vi "setUp.vi"(8 "error in (no error)":errorcluster) -> (0 "error out":errorcluster, 2 "connection ID":refnum<k5>, 3 "session":T1)   [LabVIEW 2017, in "support.lvlib"]
doc: "Initialize the library, open a connection and authenticate a session with the SSH server."
uses:
  support.lvlib
  libssh2/Session Refnum.ctl
  <vilib>/Utility/error.llb/DialogType.ctl
  libssh2/libssh2_session_handshake_tcp.vi
  libssh2/libssh2_init_default.vi
  libssh2/libssh2_session_init_ex.vi
  <vilib>/Utility/tcp.llb/TCP Get Raw Net Object.vi
  libssh2/libssh2_session_handshake_socket.vi
  libssh2/libssh2.lvlib
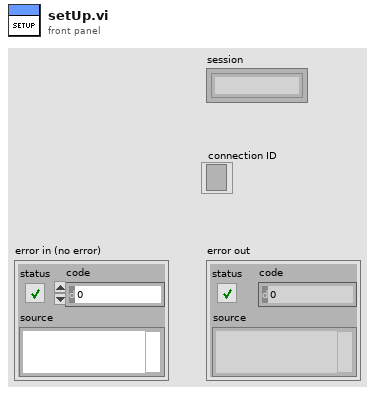
[diagram p1: front panel]
types:
  T1 = typedef "libssh2.lvlib/Session Refnum.ctl" = refnum<k1>
  T2 = typedef "DialogType.ctl" = u16
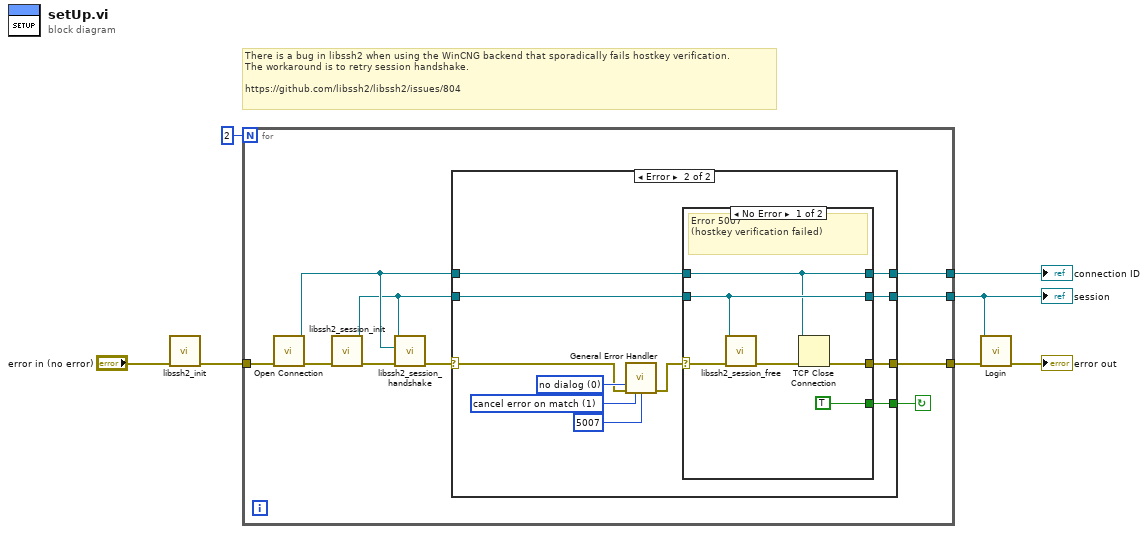
[diagram p0: block diagram]
diagram:
  # "There is a bug in libssh2 when using the WinCNG backend that sporadically fails hostkey verification.\nThe workaround is to retry session handshake.\n\nhttps://github.com/libssh2/libssh2/issues/804"
  n1 = call-poly "libssh2_init.vi"("error in (no error)"="error in (no error)") -> ("error out"=w7:errorcluster)  [unwired: 10 in]
  n2 = for {
    N: 2 -> [_]
    tunnel: w7 -> [w16]
    tunnel: [w13] -> w4
    tunnel: [w11] -> w3
    tunnel: [w9] -> w2
    stop <- w8 continue-if-true
    n3 = call "Open Connection.vi"("error in (no error)"=w16) -> ("error out"=w17:errorcluster, "connection ID"=w12:refnum<k5>)  [unwired: 9 in]
    n4 = call "libssh2_session_init.vi"("error in (no error)"=w17) -> ("error out"=w15:errorcluster, "session"=w10:T1)  [unwired: 9 in]
    n5 = call-poly "libssh2_session_handshake.vi"("error in (no error)"=w15, "tcp connection"=w12, "session"=w10) -> ("error out"=w14:errorcluster)  [unwired: 8 in]
    n6 = case shown="Error" w14 {
      selector: w14 -> [w20 w28]
      tunnel: [w20 w26] -> w13
      tunnel: w12 -> [w19 w25]
      tunnel: [w19 w24] -> w11
      tunnel: w10 -> [w18 w22]
      tunnel: [w18 w23] -> w9
      tunnel: [_ w21] -> w8
      frame No Error {
      }
      frame Error {
        w30 = T2 0 items=["no dialog", "OK message", "continue or stop message", "OK message + warnings", "continue/stop + warnings"] ("type of dialog (OK msg:1)")
        w31 = 1 items=["no exception", "cancel error on match", "set error on match"] ("[exception action] (none:0)")
        n7 = call <vilib>:"General Error Handler.vi"("type of dialog (OK msg:1)"=w30, "error in (no error)"=w28, "[exception action] (none:0)"=w31, "[exception code]"=5007 ("specific error code to clear (0: all)")) -> ("error out"=w27:errorcluster)  [unwired: 7 in, 4 out]
        n8 = case shown="No Error" w27 {
          selector: w27 -> [w36 w40]
          tunnel: [w35 w40] -> w26
          tunnel: w25 -> [w33 w39]
          tunnel: [w33 w39] -> w24
          tunnel: [w34 w38] -> w23
          tunnel: w22 -> [w34 w38]
          tunnel: [TRUE _] -> w21
          frame No Error {
            # "Error 5007\n(hostkey verification failed)"
            n9 = call "libssh2_session_free.vi"("error in (no error)"=w36, "session"=w34) -> ("error out"=w37:errorcluster)  [unwired: 9 in]
            n10 = TCP Close Connection(connection ID=w33, error in (no error)=w37) -> (error out=w35:errorcluster)  [unwired: 1 in, 1 out]
          }
          frame Error {
            # "Other errors..."
          }
        }
      }
    }
  }
  "connection ID" <- w3
  "session" <- w2
  n11 = call "Login.vi"("error in (no error)"=w4, "session"=w2) -> ("error out"=→"error out":errorcluster)  [unwired: 9 in]
